vi "Array filter - Template.vi"() -> ()   [LabVIEW 2012]
panel:
  out "Array 4":variant[](array[variant])
  out "Array 3":variant[](array[variant])
  in  "Boolean Input":bool[](array[boolean])
  in  "Array Input":variant[](array[variant])
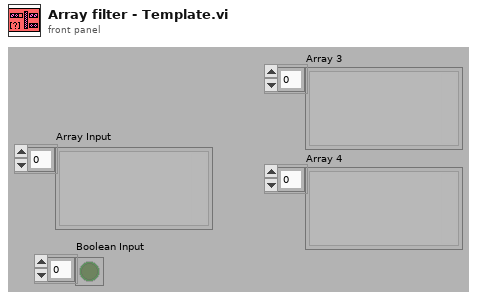
[diagram p1: front panel]
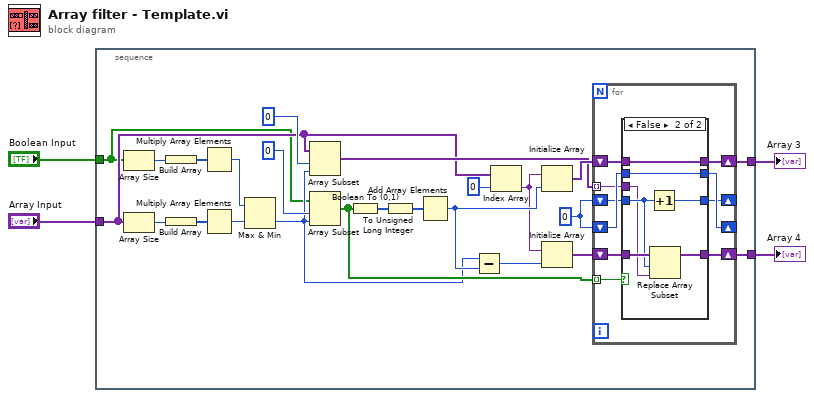
[diagram p0: block diagram]
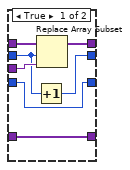
[diagram p2: hidden frame]
diagram:
  n1 = stacked-sequence {
    tunnel: "Boolean Input" -> [w8]
    tunnel: "Array Input" -> [w9]
    tunnel: [w19] -> w2
    tunnel: [w18] -> w1
    frame #0 {
      w20 = 0
      n2 = Array Size(array=w8) -> (size(s)=w17:i32)
      n3 = Array Size(array=w9) -> (size(s)=w16:i32)
      n4 = Build Array(w17) -> (w7:i32[])
      n5 = Build Array(w16) -> (w6:i32[])
      n6 = Multiply Array Elements(1:w7) -> (0:w14:i32)
      n7 = Multiply Array Elements(1:w6) -> (0:w15:i32)
      n8 = Max & Min(x=w14, y=w15) -> (min(x,y)=w12:i32)  [unwired: 1 out]
      n9 = Array Subset(array=w9, index=0, length=w12) -> (w10:variant[])
      n10 = Array Subset(array=w8, index=0, length=w12) -> (w21:bool[])
      n11 = Boolean To (0,1)(Boolean=w21) -> (0, 1=w28:i16[])
      n12 = To Unsigned Long Integer(number=w28) -> (unsigned 32bit integer=w5:u32[])
      n13 = Add Array Elements(numeric array=w5) -> (sum=w25:u32)
      n14 = Subtract(x=w12, y=w25) -> (x-y=w24:u32)
      n15 = Index Array(array=w9, index=0) -> (element=w11:variant)
      n16 = Initialize Array(w11, w25) -> (w23:variant[])
      n17 = Initialize Array(w11, w24) -> (w22:variant[])
      n18 = for {
        shift-right: [w37] -> w19
        shift-left: w23 -> [w36]
        shift-right: [w31] -> w18
        shift-left: w22 -> [w32]
        tunnel: w21 -> [w38] mode=indexing
        shift-right: [w33] -> _
        shift-left: w20 -> [w35]
        shift-right: [w29] -> _
        shift-left: w20 -> [w30]
        tunnel: w10 -> [w34] mode=indexing
        n19 = case shown="False" w38 {
          tunnel: [w41 w52] -> w37
          tunnel: w36 -> [w45 w52]
          tunnel: w35 -> [w43 w47]
          tunnel: w34 -> [w44 w46]
          tunnel: [w42 w47] -> w33
          tunnel: w32 -> [w39 w51]
          tunnel: [w39 w50] -> w31
          tunnel: w30 -> [w40 w49]
          tunnel: [w40 w48] -> w29
          frame True {
            n20 = Increment(x=w43) -> (x+1=w42:i32)
            n21 = Replace Array Subset(array=w45, new element=w44, index=w43) -> (w41:variant[])
          }
          frame False {
            n22 = Increment(x=w49) -> (x+1=w48:i32)
            n23 = Replace Array Subset(array=w51, new element=w46, index=w49) -> (w50:variant[])
          }
        }
      }
    }
  }
  "Array 3" <- w2
  "Array 4" <- w1
